vi "RemoteVI Check Parse Arguments.vi"() -> (4 "labels":string[](array[string]), 6 "expected":string[](array[string]), 8 "actual":string[](array[string]), 10 "failures":i32)   [LabVIEW 2020]
doc: "Test support, generated by tests/caraya/build.py from tests/vectors/server-app.json (parseArgs) - do not edit. Calls RemoteVI Parse Arguments.vi once per vector: args as in the vector; the options are rendered share|port|token|whole network|view only|landing port with T or F. Outputs, one element per vector: labels (the vector's name), expected (rendered from the vector), actual (the VI's result rendered the same way), and failures, the number of vectors whose expected and actual differ."
uses:
  source/RemoteVI.lvlib
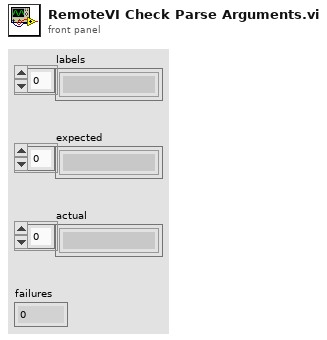
[diagram p1: front panel]
types:
  T1 = cluster{"name":string, "args":string[], "expect":string}[]
  T2 = cluster{"share":string, "port":u16, "token":string, "whole network":bool, "view only":bool, "landing port":u16}
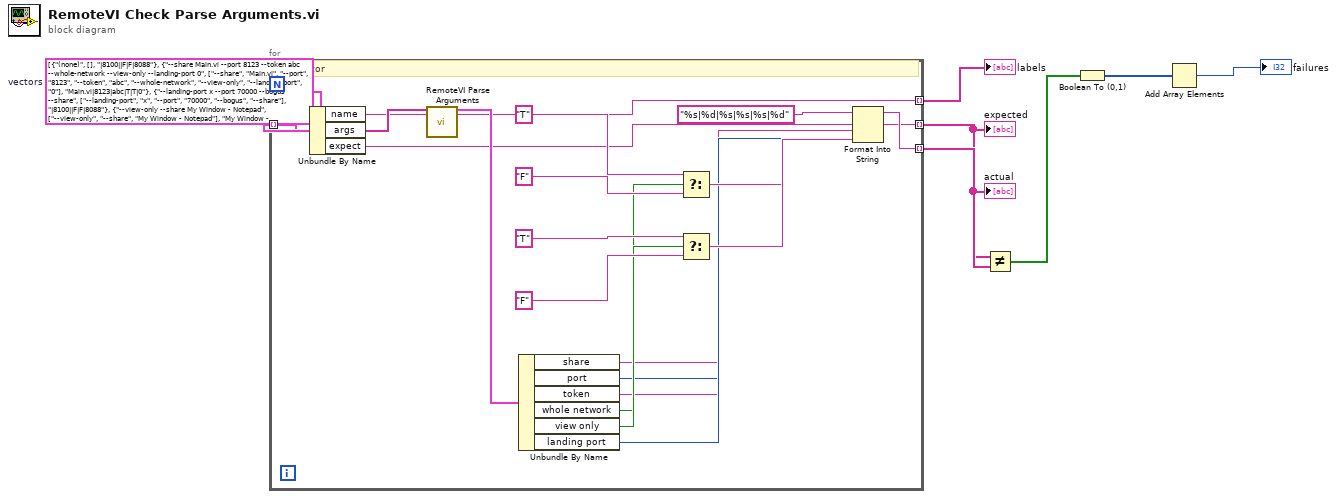
[diagram p0: block diagram]
diagram:
  w1 = T1 [{"name"="(none)", "args"=[], "expect"="|8100||F|F|8088"}, {"name"="--share Main.vi --port 8123 --token abc --whole-network --view-only --landing-port 0", "args"=["--share", "Main.vi", "--port", "8123", "--token", "abc", "--whole-network", "--view-only", "--landing-port", "0"], "expect"="Main.vi|8123|abc|T|T|0"}, {"name"="--landing-port x --port 70000 --bogus --share", "args"=["--landing-port", "x", "--port", "70000", "--bogus", "--share"], "expect"="|8100||F|F|8088"}, {"name"="--view-only --share My Window - Notepad", "args"=["--view-only", "--share", "My Window - Notepad"], "expect"="My Window - Notepad|8100||F|T|8088"}]  # vectors
  n1 = for {
    tunnel: w1 -> [w8] mode=indexing
    tunnel: [w9] -> w2 mode=indexing
    tunnel: [w11] -> w3 mode=indexing
    tunnel: [w26] -> w4 mode=indexing
    # "One vector"
    n2 = Unbundle By Name(w8) -> ("name"=w9:string, "args"=w10:string[], "expect"=w11:string)
    n3 = call "RemoteVI Parse Arguments.vi"("args"=w10) -> ("options"=w12:T2)  [unwired: 14 in]
    n4 = Unbundle By Name(w12) -> ("share"=w13:string, "port"=w14:u16, "token"=w15:string, "whole network"=w16:bool, "view only"=w17:bool, "landing port"=w18:u16)
    n5 = Select(t="T", s=w16, f="F") -> (s? t:f=w21:string)
    n6 = Select(t="T", s=w17, f="F") -> (s? t:f=w24:string)
    n7 = Format Into String(format string="%s|%d|%s|%s|%s|%d", w13, w14, w15, w21, w24, w18) -> (resulting string=w26:string)  [unwired: 2 in, 1 out]
  }
  "labels" <- w2
  "expected" <- w3
  "actual" <- w4
  n8 = Not Equal?(x=w3, y=w4) -> (x != y?=w5:bool[])
  n9 = Boolean To (0,1)(Boolean=w5) -> (0, 1=w6:i16[])
  n10 = Add Array Elements(numeric array=w6) -> (sum=→"failures":i16)
